vi "onTestExecution.vi"(6 "timeout (2000 ms)":i32=2000, 7 "Name":string, 8 "error in (no error)":errorcluster, 11 "Unit Tests for Runner in":refnum<class "Unit Tests for Runner.lvclass">) -> (0 "error out":errorcluster, 3 "Unit Tests for Runner out":refnum<class "Unit Tests for Runner.lvclass">)   [LabVIEW 2020, in "Unit Tests for Runner.lvclass"]
uses:
  Unit Tests for Runner.lvclass
  classes/Test Runner/Test Runner.lvclass
  classes/Test/Test.lvclass
  classes/Assert/Assert.lvclass
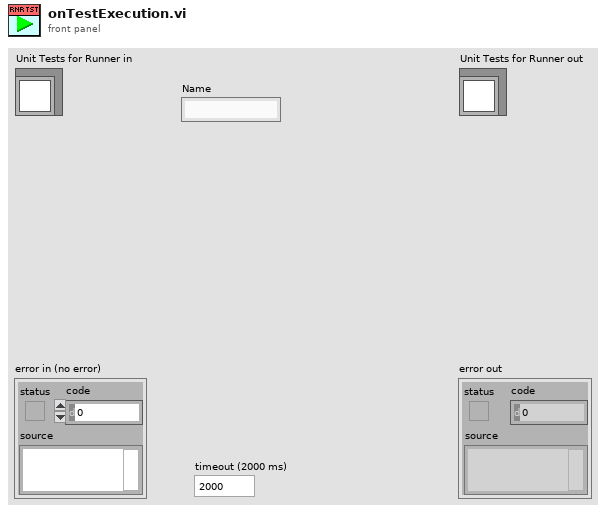
[diagram p1: front panel]
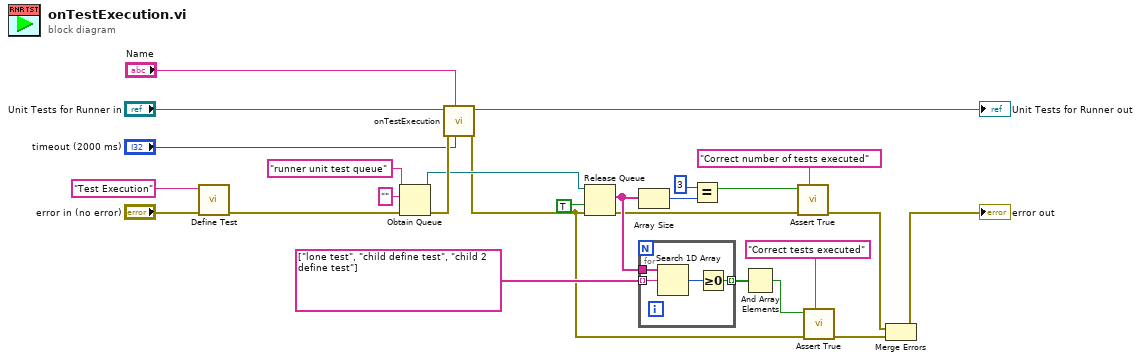
[diagram p0: block diagram]
diagram:
  n1 = call "Define Test.vi"("error in (no error)"="error in (no error)", "Label (VI Title)"="Test Execution" ("name (unnamed)")) -> ("error out"=w2:errorcluster)  [unwired: 8 in, 1 out]
  n2 = Obtain Queue(name (unnamed)="runner unit test queue", element data type="", error in (no error)=w2) -> (queue out=w7:refnum<queue>, error out=w21:errorcluster)  [unwired: 2 in, 1 out]
  n3 = call-parent "onTestExecution.vi"("timeout (2000 ms)"="timeout (2000 ms)", "Name"="Name", "error in (no error)"=w21, "Test Runner in"="Unit Tests for Runner in") -> ("error out"=w4:errorcluster, "Test Runner out"=→"Unit Tests for Runner out":refnum<class "Unit Tests for Runner.lvclass">)  [unwired: 6 in]
  n4 = Release Queue(queue=w7, force destroy? (F)=TRUE, error in (no error)=w4) -> (remaining elements=w18:string[], error out=w14:errorcluster)  [unwired: 1 out]
  n5 = Array Size(array=w18) -> (size(s)=w17:i32)
  n6 = for {
    tunnel: w18 -> [w30]
    tunnel: string[] ["lone test", "child define test", "child 2 define test"] -> [w29] mode=indexing
    tunnel: [w27] -> w13 mode=indexing
    n7 = Search 1D Array(1D array=w30, element=w29) -> (index of element=w28:i32)  [unwired: 1 in]
    n8 = Greater Or Equal To 0?(x=w28) -> (x >= 0?=w27:bool)
  }
  n9 = Equal?(x=3, y=w17) -> (x = y?=w9:bool)
  n10 = And Array Elements(Boolean array=w13) -> (logical AND=w10:bool)
  n11 = call "Assert True.vi"("Label"="Correct number of tests executed", "error in (no error)"=w14, "True?"=w9) -> ("error out"=w8:errorcluster)  [unwired: 7 in, 1 out]
  n12 = call "Assert True.vi"("Label"="Correct tests executed", "error in (no error)"=w4, "True?"=w10) -> ("error out"=w11:errorcluster)  [unwired: 7 in, 1 out]
  n13 = Merge Errors(w8, w11) -> (→"error out":errorcluster)
